vi "Test_Configurable_Parse_Caraya.vi"(8 "error in":errorcluster) -> (0 "error out":errorcluster)   [LabVIEW 2026]
doc: "Caraya tests of the configurable sequence parser, the rig IO list reader and the name and type validator."
uses:
  <vilib>/addons/_JKI Toolkits/Caraya/classes/Test/Test.lvclass
  <vilib>/addons/_JKI Toolkits/Caraya/classes/Assert/Assert.lvclass
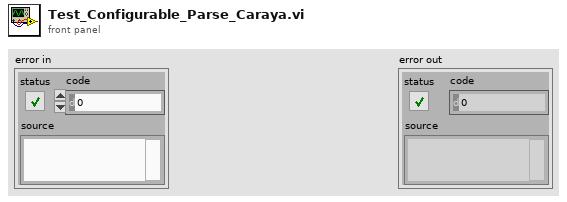
[diagram p1: front panel]
types:
  T1 = cluster{"sequence_id":string, "description":string, "rig_config":string, "steps":cluster{"step_no":i32, "step_name":string, "interlock_status":string, "pre_delay_ms":dbl, "post_delay_ms":dbl, "timeout_ms":dbl, "popup":cluster{"enabled":bool, "message":string, "type":string, "timeout_ms":dbl}, "retest":cluster{"enabled":bool, "popup":bool, "popup_message":string, "condition":string, "goto_step_no":i32}, "log":cluster{"peak":bool, "average":bool, "event":bool}, "actions":cluster{"do":cluster{"name":string, "on":bool, "mode":string}[], "ao":cluster{"name":string, "value":dbl, "mode":string}[], "misc_write":cluster{"name":string, "on":bool}[], "call":string[]}, "checks":cluster{"di_high":cluster{"and":string[], "or":string[]}, "di_low":cluster{"and":string[], "or":string[]}, "misc_high":cluster{"and":string[], "or":string[]}, "misc_low":cluster{"and":string[], "or":string[]}, "t0_high":cluster{"and":cluster{"name":string, "min":dbl, "max":dbl}[], "or":cluster{"name":string, "min":dbl, "max":dbl}[]}, "t0_low":cluster{"and":cluster{"name":string, "min":dbl, "max":dbl}[], "or":cluster{"name":string, "min":dbl, "max":dbl}[]}, "misc_compare":cluster{"name":string, "compare_with":string, "comparison":string, "tolerance":dbl}[]}}[]}
  T2 = cluster{"step_no":i32, "step_name":string, "interlock_status":string, "pre_delay_ms":dbl, "post_delay_ms":dbl, "timeout_ms":dbl, "popup":cluster{"enabled":bool, "message":string, "type":string, "timeout_ms":dbl}, "retest":cluster{"enabled":bool, "popup":bool, "popup_message":string, "condition":string, "goto_step_no":i32}, "log":cluster{"peak":bool, "average":bool, "event":bool}, "actions":cluster{"do":cluster{"name":string, "on":bool, "mode":string}[], "ao":cluster{"name":string, "value":dbl, "mode":string}[], "misc_write":cluster{"name":string, "on":bool}[], "call":string[]}, "checks":cluster{"di_high":cluster{"and":string[], "or":string[]}, "di_low":cluster{"and":string[], "or":string[]}, "misc_high":cluster{"and":string[], "or":string[]}, "misc_low":cluster{"and":string[], "or":string[]}, "t0_high":cluster{"and":cluster{"name":string, "min":dbl, "max":dbl}[], "or":cluster{"name":string, "min":dbl, "max":dbl}[]}, "t0_low":cluster{"and":cluster{"name":string, "min":dbl, "max":dbl}[], "or":cluster{"name":string, "min":dbl, "max":dbl}[]}, "misc_compare":cluster{"name":string, "compare_with":string, "comparison":string, "tolerance":dbl}[]}}[]
  T3 = cluster{"step_no":i32, "step_name":string, "interlock_status":string, "pre_delay_ms":dbl, "post_delay_ms":dbl, "timeout_ms":dbl, "popup":cluster{"enabled":bool, "message":string, "type":string, "timeout_ms":dbl}, "retest":cluster{"enabled":bool, "popup":bool, "popup_message":string, "condition":string, "goto_step_no":i32}, "log":cluster{"peak":bool, "average":bool, "event":bool}, "actions":cluster{"do":cluster{"name":string, "on":bool, "mode":string}[], "ao":cluster{"name":string, "value":dbl, "mode":string}[], "misc_write":cluster{"name":string, "on":bool}[], "call":string[]}, "checks":cluster{"di_high":cluster{"and":string[], "or":string[]}, "di_low":cluster{"and":string[], "or":string[]}, "misc_high":cluster{"and":string[], "or":string[]}, "misc_low":cluster{"and":string[], "or":string[]}, "t0_high":cluster{"and":cluster{"name":string, "min":dbl, "max":dbl}[], "or":cluster{"name":string, "min":dbl, "max":dbl}[]}, "t0_low":cluster{"and":cluster{"name":string, "min":dbl, "max":dbl}[], "or":cluster{"name":string, "min":dbl, "max":dbl}[]}, "misc_compare":cluster{"name":string, "compare_with":string, "comparison":string, "tolerance":dbl}[]}}
  T4 = cluster{"enabled":bool, "message":string, "type":string, "timeout_ms":dbl}
  T5 = cluster{"di_high":cluster{"and":string[], "or":string[]}, "di_low":cluster{"and":string[], "or":string[]}, "misc_high":cluster{"and":string[], "or":string[]}, "misc_low":cluster{"and":string[], "or":string[]}, "t0_high":cluster{"and":cluster{"name":string, "min":dbl, "max":dbl}[], "or":cluster{"name":string, "min":dbl, "max":dbl}[]}, "t0_low":cluster{"and":cluster{"name":string, "min":dbl, "max":dbl}[], "or":cluster{"name":string, "min":dbl, "max":dbl}[]}, "misc_compare":cluster{"name":string, "compare_with":string, "comparison":string, "tolerance":dbl}[]}
diagram:
  w5 = "empty steps error 5001"  # label empty steps error 5001
  w6 = 5001  # 5001
  w10 = "{\"sequence_id\":\"E\",\"description\":\"\",\"rig_config\":\"\",\"steps\":[]}"  # json empty
  w14 = "wrong type rejected"  # label wrong type rejected
  w15 = "OIL LEVEL OK is not a valid IO for this use"  # wrong msg
  w19 = "{\"sequence_id\":\"X\",\"description\":\"\",\"rig_config\":\"\",\"steps\":[{\"step_no\":2,\"step_name\":\"Lubrication System: Delay Only\",\"interlock_status\":\"\",\"pre_delay_ms\":2000,\"post_delay_ms\":0,\"timeout_ms\":0,\"popup\":{\"enabled\":false,\"message\":\"\",\"type\":\"OK\",\"timeout_ms\":0},\"retest\":{\"enabled\":false,\"popup\":false,\"popup_message\":\"\",\"condition\":\"\",\"goto_step_no\":0},\"log\":{\"peak\":false,\"average\":false,\"event\":false},\"actions\":{\"do\":[{\"name\":\"OIL LEVEL OK\",\"on\":true,\"mode\":\"FROM_IO\"}],\"ao\":[],\"misc_write\":[],\"call\":[]},\"checks\":{\"di_high\":{\"and\":[],\"or\":[]},\"di_low\":{\"and\":[],\"or\":[]},\"misc_high\":{\"and\":[],\"or\":[]},\"misc_low\":{\"and\":[],\"or\":[]},\"t0_high\":{\"and\":[],\"or\":[]},\"t0_low\":{\"and\":[],\"or\":[]},\"misc_compare\":[]}}]}"  # json wrong
  w23 = "unknown name error 5002"  # label unknown name error 5002
  w24 = 5002  # 5002
  w30 = "unknown name rejected"  # label unknown name rejected
  w31 = "NOPE is not a valid IO for this use"  # unknown msg
  w34 = "{\"sequence_id\":\"X\",\"description\":\"\",\"rig_config\":\"\",\"steps\":[{\"step_no\":2,\"step_name\":\"Lubrication System: Delay Only\",\"interlock_status\":\"\",\"pre_delay_ms\":2000,\"post_delay_ms\":0,\"timeout_ms\":0,\"popup\":{\"enabled\":false,\"message\":\"\",\"type\":\"OK\",\"timeout_ms\":0},\"retest\":{\"enabled\":false,\"popup\":false,\"popup_message\":\"\",\"condition\":\"\",\"goto_step_no\":0},\"log\":{\"peak\":false,\"average\":false,\"event\":false},\"actions\":{\"do\":[],\"ao\":[],\"misc_write\":[],\"call\":[]},\"checks\":{\"di_high\":{\"and\":[\"NOPE\"],\"or\":[]},\"di_low\":{\"and\":[],\"or\":[]},\"misc_high\":{\"and\":[],\"or\":[]},\"misc_low\":{\"and\":[],\"or\":[]},\"t0_high\":{\"and\":[],\"or\":[]},\"t0_low\":{\"and\":[],\"or\":[]},\"misc_compare\":[]}}]}"  # json unknown
  w38 = "sample validate no error"  # label sample validate no error
  w45 = "sample validates"  # label sample validates
  w46 = ""  # no problem
  w52 = "step 2 checks empty"  # label step 2 checks empty
  w53 = 0  # zero
  w61 = "step 2 popup off"  # label step 2 popup off
  w67 = "step 2 pre delay read"  # label step 2 pre delay read
  w68 = 2000.0  # two thousand
  w74 = "step 1 first di_high item"  # label step 1 first di_high item
  w75 = "OIL LEVEL OK"  # oil
  w77 = 0  # index 5035
  w84 = "step 1 popup enabled"  # label step 1 popup enabled
  w89 = 1  # index 5024
  w91 = 0  # index 5021
  w95 = "parse sample has 2 steps"  # label parse sample has 2 steps
  w96 = 2  # two
  w101 = "parse sample has no error"  # label parse sample has no error
  w104 = "{\"sequence_id\":\"CONFIGURABLE_SAMPLE\",\"description\":\"Sample of the configurable step format. Draft: the executor does not read this format yet.\",\"rig_config\":\"../rigs/configurable_sim.json\",\"steps\":[{\"step_no\":1,\"step_name\":\"Lubrication System: Pump ON\",\"interlock_status\":\"Waiting for pump running feedback\",\"pre_delay_ms\":500,\"post_delay_ms\":1000,\"timeout_ms\":10000,\"popup\":{\"enabled\":true,\"message\":\"Confirm oil level\",\"type\":\"OK\",\"timeout_ms\":0},\"retest\":{\"enabled\":false,\"popup\":false,\"popup_message\":\"\",\"condition\":\"\",\"goto_step_no\":0},\"log\":{\"peak\":false,\"average\":false,\"event\":true},\"actions\":{\"do\":[{\"name\":\"LUB PUMP\",\"on\":true,\"mode\":\"FROM_IO\"}],\"ao\":[{\"name\":\"PRESSURE SETPOINT\",\"value\":20.0,\"mode\":\"FROM_IO\"}],\"misc_write\":[],\"call\":[]},\"checks\":{\"di_high\":{\"and\":[\"OIL LEVEL OK\",\"LUB PUMP RUNNING\"],\"or\":[]},\"di_low\":{\"and\":[\"EMERGENCY STOP\"],\"or\":[]},\"misc_high\":{\"and\":[],\"or\":[]},\"misc_low\":{\"and\":[],\"or\":[]},\"t0_high\":{\"and\":[{\"name\":\"LUB PRESSURE\",\"min\":18.0,\"max\":22.0}],\"or\":[]},\"t0_low\":{\"and\":[],\"or\":[]},\"misc_compare\":[]}},{\"step_no\":2,\"step_name\":\"Lubrication System: Delay Only\",\"interlock_status\":\"\",\"pre_delay_ms\":2000,\"post_delay_ms\":0,\"timeout_ms\":0,\"popup\":{\"enabled\":false,\"message\":\"\",\"type\":\"OK\",\"timeout_ms\":0},\"retest\":{\"enabled\":false,\"popup\":false,\"popup_message\":\"\",\"condition\":\"\",\"goto_step_no\":0},\"log\":{\"peak\":false,\"average\":false,\"event\":false},\"actions\":{\"do\":[],\"ao\":[],\"misc_write\":[],\"call\":[]},\"checks\":{\"di_high\":{\"and\":[],\"or\":[]},\"di_low\":{\"and\":[],\"or\":[]},\"misc_high\":{\"and\":[],\"or\":[]},\"misc_low\":{\"and\":[],\"or\":[]},\"t0_high\":{\"and\":[],\"or\":[]},\"t0_low\":{\"and\":[],\"or\":[]},\"misc_compare\":[]}}]}"  # json sample
  w39 = FALSE  # false
  w85 = TRUE  # true
  w105 = "{\"rig_id\":\"CONFIGURABLE_SIM\",\"description\":\"Sample rig for the configurable step format. Draft: the executor does not read this format yet.\",\"plugin_class\":\"../../plugins/VTU Sim Rig/VTU Sim Rig.lvclass\",\"channels\":[{\"name\":\"EMERGENCY STOP\",\"type\":\"DI\"},{\"name\":\"OIL LEVEL OK\",\"type\":\"DI\"},{\"name\":\"LUB PUMP RUNNING\",\"type\":\"DI\"},{\"name\":\"LUB PUMP\",\"type\":\"DO\"},{\"name\":\"PRESSURE SETPOINT\",\"type\":\"AO\",\"unit\":\"bar\",\"min\":0,\"max\":250},{\"name\":\"LUB PRESSURE\",\"type\":\"AI\",\"unit\":\"bar\",\"min\":0,\"max\":250},{\"name\":\"OPERATOR READY\",\"type\":\"MISC_BOOL\"}]}"  # rig json
  w9 = errorcluster {"status"=FALSE, "code"=0, "source"=""}  # no error
  n1 = call "Parse Configurable Sequence.vi"("error in"=w9, "JSON string"=w10) -> ("error out"=w8:errorcluster)  [unwired: 8 in, 1 out]
  n2 = call "Parse Configurable Sequence.vi"("error in"=w9, "JSON string"=w19) -> ("Configurable Sequence"=w18:T1)  [unwired: 8 in, 1 out]
  n3 = call "Parse Configurable Sequence.vi"("error in"=w9, "JSON string"=w34) -> ("Configurable Sequence"=w33:T1)  [unwired: 8 in, 1 out]
  n4 = call "Parse Rig IO List.vi"("error in"=w9, "JSON string"=w105) -> ("IO List"=w17:cluster{"name":string, "type":string}[])  [unwired: 8 in, 1 out]
  n5 = call "Parse Configurable Sequence.vi"("error in"=w9, "JSON string"=w104) -> ("error out"=w103:errorcluster, "Configurable Sequence"=w48:T1)  [unwired: 8 in]
  n6 = Unbundle By Name(w103) -> ("status"=w102:bool)
  n7 = Unbundle By Name(w8) -> ("code"=w7:i32)
  n8 = Unbundle By Name(w48) -> ("steps"=w90:T2)
  n9 = call "Validate Configurable Sequence.vi"("error in"=w9, "IO List"=w17, "Configurable Sequence"=w18) -> ("problem"=w16:string)  [unwired: 7 in, 1 out]
  n10 = call "Validate Configurable Sequence.vi"("error in"=w9, "IO List"=w17, "Configurable Sequence"=w33) -> ("error out"=w26:errorcluster, "problem"=w32:string)  [unwired: 7 in]
  n11 = call "Validate Configurable Sequence.vi"("error in"=w9, "IO List"=w17, "Configurable Sequence"=w48) -> ("error out"=w41:errorcluster, "problem"=w47:string)  [unwired: 7 in]
  n12 = Unbundle By Name(w41) -> ("status"=w40:bool)
  n13 = Unbundle By Name(w26) -> ("code"=w25:i32)
  n14 = Array Size(array=w90) -> (size(s)=w97:i32)
  n15 = To Variant(anything=w16) -> (Variant=w12:variant)
  n16 = To Variant(anything=w32) -> (Variant=w28:variant)
  n17 = To Variant(anything=w47) -> (Variant=w43:variant)
  n18 = Index Array(array=w90, index=w91) -> (element=w88:T3)
  n19 = Unbundle By Name(w88) -> ("popup"=w87:T4, "checks"=w80:T5)
  n20 = call <vilib>:"Define Test.vi"("error in (no error)"="error in") -> ("error out"=w100:errorcluster)  [unwired: 9 in, 1 out]
  n21 = To Variant(anything=w39) -> (Variant=w98:variant)
  n22 = To Variant(anything=w102) -> (Variant=w99:variant)
  n23 = Unbundle By Name(w87) -> ("enabled"=w86:bool)
  n24 = Unbundle By Name(w80) -> ("di_high"=w79:cluster{"and":string[], "or":string[]})
  n25 = call <vilib>:"Assert Equal Value_Variant.vi"("Label"=w101, "error in (no error)"=w100, "Actual"=w99, "Expected"=w98) -> ("error out"=w94:errorcluster)  [unwired: 6 in, 1 out]
  n26 = To Variant(anything=w97) -> (Variant=w93:variant)
  n27 = Unbundle By Name(w79) -> ("and"=w78:string[])
  n28 = To Variant(anything=w39) -> (Variant=w35:variant)
  n29 = To Variant(anything=w40) -> (Variant=w36:variant)
  n30 = To Variant(anything=w39) -> (Variant=w58:variant)
  n31 = To Variant(anything=w86) -> (Variant=w82:variant)
  n32 = To Variant(anything=w96) -> (Variant=w92:variant)
  n33 = call <vilib>:"Assert Equal Value_Variant.vi"("Label"=w95, "error in (no error)"=w94, "Actual"=w93, "Expected"=w92) -> ("error out"=w83:errorcluster)  [unwired: 6 in, 1 out]
  n34 = Index Array(array=w90, index=w89) -> (element=w70:T3)
  n35 = Unbundle By Name(w70) -> ("pre_delay_ms"=w69:dbl, "popup"=w63:T4, "checks"=w57:T5)
  n36 = Index Array(array=w78, index=w77) -> (element=w76:string)
  n37 = To Variant(anything=w85) -> (Variant=w81:variant)
  n38 = Unbundle By Name(w63) -> ("enabled"=w62:bool)
  n39 = Unbundle By Name(w57) -> ("di_high"=w56:cluster{"and":string[], "or":string[]})
  n40 = call <vilib>:"Assert Equal Value_Variant.vi"("Label"=w84, "error in (no error)"=w83, "Actual"=w82, "Expected"=w81) -> ("error out"=w73:errorcluster)  [unwired: 6 in, 1 out]
  n41 = To Variant(anything=w75) -> (Variant=w71:variant)
  n42 = To Variant(anything=w76) -> (Variant=w72:variant)
  n43 = Unbundle By Name(w56) -> ("and"=w55:string[])
  n44 = call <vilib>:"Assert Equal Value_Variant.vi"("Label"=w74, "error in (no error)"=w73, "Actual"=w72, "Expected"=w71) -> ("error out"=w66:errorcluster)  [unwired: 6 in, 1 out]
  n45 = To Variant(anything=w62) -> (Variant=w59:variant)
  n46 = To Variant(anything=w68) -> (Variant=w64:variant)
  n47 = To Variant(anything=w69) -> (Variant=w65:variant)
  n48 = Array Size(array=w55) -> (size(s)=w54:i32)
  n49 = call <vilib>:"Assert Equal Value_Variant.vi"("Label"=w67, "error in (no error)"=w66, "Actual"=w65, "Expected"=w64) -> ("error out"=w60:errorcluster)  [unwired: 6 in, 1 out]
  n50 = call <vilib>:"Assert Equal Value_Variant.vi"("Label"=w61, "error in (no error)"=w60, "Actual"=w59, "Expected"=w58) -> ("error out"=w51:errorcluster)  [unwired: 6 in, 1 out]
  n51 = To Variant(anything=w54) -> (Variant=w50:variant)
  n52 = To Variant(anything=w53) -> (Variant=w49:variant)
  n53 = call <vilib>:"Assert Equal Value_Variant.vi"("Label"=w52, "error in (no error)"=w51, "Actual"=w50, "Expected"=w49) -> ("error out"=w44:errorcluster)  [unwired: 6 in, 1 out]
  n54 = To Variant(anything=w46) -> (Variant=w42:variant)
  n55 = call <vilib>:"Assert Equal Value_Variant.vi"("Label"=w45, "error in (no error)"=w44, "Actual"=w43, "Expected"=w42) -> ("error out"=w37:errorcluster)  [unwired: 6 in, 1 out]
  n56 = call <vilib>:"Assert Equal Value_Variant.vi"("Label"=w38, "error in (no error)"=w37, "Actual"=w36, "Expected"=w35) -> ("error out"=w29:errorcluster)  [unwired: 6 in, 1 out]
  n57 = To Variant(anything=w31) -> (Variant=w27:variant)
  n58 = call <vilib>:"Assert Equal Value_Variant.vi"("Label"=w30, "error in (no error)"=w29, "Actual"=w28, "Expected"=w27) -> ("error out"=w22:errorcluster)  [unwired: 6 in, 1 out]
  n59 = To Variant(anything=w24) -> (Variant=w20:variant)
  n60 = To Variant(anything=w25) -> (Variant=w21:variant)
  n61 = call <vilib>:"Assert Equal Value_Variant.vi"("Label"=w23, "error in (no error)"=w22, "Actual"=w21, "Expected"=w20) -> ("error out"=w13:errorcluster)  [unwired: 6 in, 1 out]
  n62 = To Variant(anything=w15) -> (Variant=w11:variant)
  n63 = call <vilib>:"Assert Equal Value_Variant.vi"("Label"=w14, "error in (no error)"=w13, "Actual"=w12, "Expected"=w11) -> ("error out"=w4:errorcluster)  [unwired: 6 in, 1 out]
  n64 = To Variant(anything=w6) -> (Variant=w2:variant)
  n65 = To Variant(anything=w7) -> (Variant=w3:variant)
  n66 = call <vilib>:"Assert Equal Value_Variant.vi"("Label"=w5, "error in (no error)"=w4, "Actual"=w3, "Expected"=w2) -> ("error out"=→"error out":errorcluster)  [unwired: 6 in, 1 out]
